vi "VIH Dialog - VI Terminals - Conpane Image.vi"(8 "error in":errorcluster, 9 "Conpane Image":T1, 10 "Original VI Name":string, 11 "VI Reference":refnum<vi>) -> (0 "error out":errorcluster, 1 "Rectangle":T2, 2 "image":picture, 3 "dup VI Reference":refnum<vi>)   [LabVIEW 2014]
doc: "::: VI Helpeks :::\nCopyright (c) 2000-2026 Konstantin Shifershteyn. All rights reserved."
uses:
  <vilib>/picture/picture.llb/imagedata.ctl
  <vilib>/Utility/miscctls.llb/LVPointTypeDef.ctl
panel:
  in  "Default Image":picture
  in  "Font prototype":string
  # "VI Helpeks\nCopyright (c) 2012-2026 Konstantin Shifershteyn"
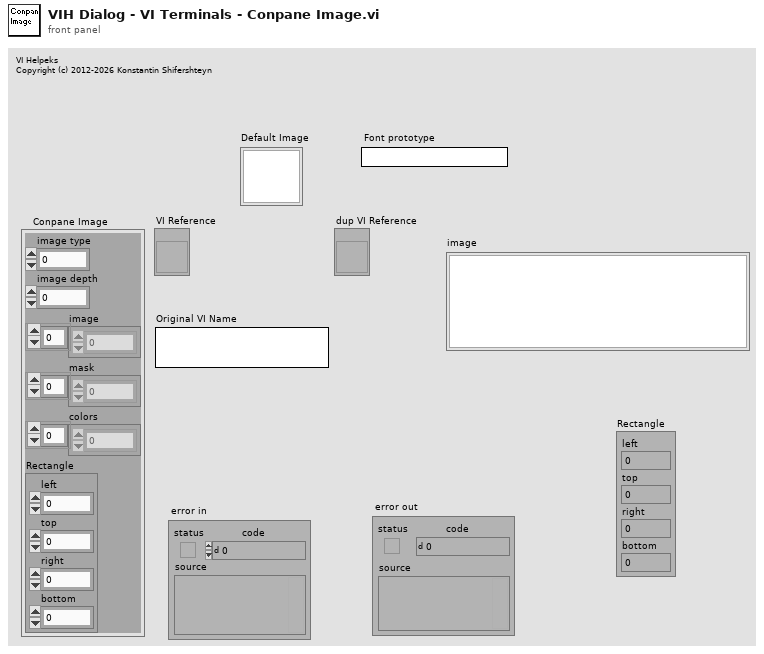
[diagram p1: front panel]
types:
  T1 = typedef "imagedata.ctl" = cluster{"image type":i32, "image depth":i32, "image":u8[], "mask":u8[], "colors":u32[], "Rectangle":cluster{"left":i16, "top":i16, "right":i16, "bottom":i16}}
  T2 = cluster{"left":i16, "top":i16, "right":i16, "bottom":i16}
  T3 = cluster{"Width":i16, "Style":enum32{"Solid", "Dash", "Dot", "DashDot", "DashDotDot"}}
  T4 = cluster{"Width":u16, "Style":enum32{"Solid", "Dash", "Dot", "DashDot", "DashDotDot"}}
  T5 = cluster{"Font Name:":string, "Size":i16, "Strikeout?":bool, "Italic?":bool, "Underline?":bool, "Outline?":bool, "Shadow?":bool, "Bold?":bool}
  T6 = enum16{"User-specified Font", "Application Font", "System Font", "Dialog Font"}
  T7 = typedef "LVPointTypeDef.ctl" = cluster{"Horizontal":i16, "Vertical":i16}
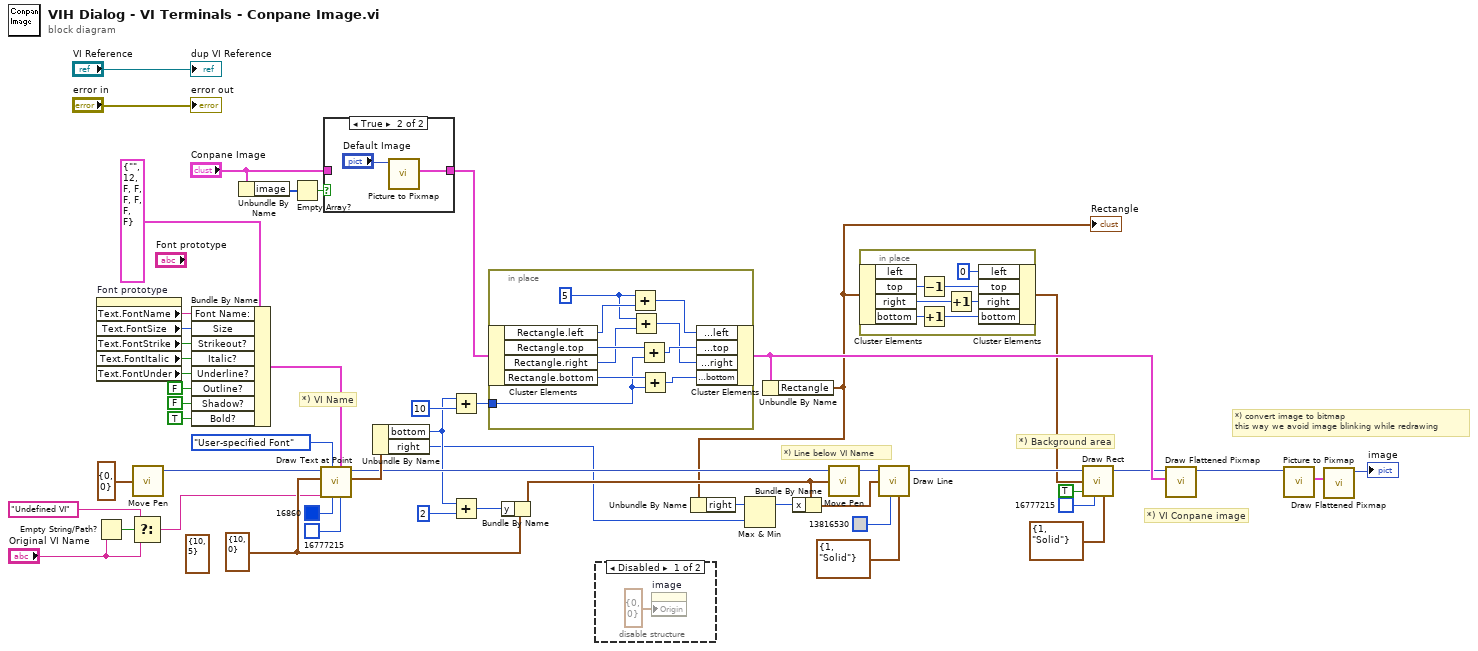
[diagram p0: block diagram]
diagram:
  (unwired) cluster{"x":i16, "y":i16} {"x"=10, "y"=5} ("origin")
  w24 = cluster{"x":i16, "y":i16} {"x"=10, "y"=0} ("origin")
  # "*) Background area"
  # "*) convert image to bitmap\nthis way we avoid image blinking while redrawing"
  # "*) VI Name"
  # "*) Line below VI Name"
  # "*) VI Conpane image"
  n1 = Empty String/Path?(string/path="Original VI Name") -> (empty?=w7:bool)
  n2 = property on="Font prototype" class="Str"() -> ("Text.FontName"=w41:string, "Text.FontSize"=w42:u32, "Text.FontStrike"=w43:bool, "Text.FontItalic"=w44:bool, "Text.FontUnder"=w45:bool)  [unwired: 2 in, 2 out]
  n3 = Select(t="Undefined VI", s=w7, f="Original VI Name") -> (s? t:f=w5:string)
  n4 = call <vilib>:"Move Pen.vi"("new position"=cluster{"x":i16, "y":i16} {"x"=0, "y"=0} ("origin")) -> ("new picture"=w19:picture)  [unwired: 4 in]
  n5 = Bundle By Name(cluster=T5 {"Font Name:"="", "Size"=12, "Strikeout?"=FALSE, "Italic?"=FALSE, "Underline?"=FALSE, "Outline?"=FALSE, "Shadow?"=FALSE, "Bold?"=FALSE} ("[user-specified font]"), "Font Name:"=w41, "Size"=w42, "Strikeout?"=w43, "Italic?"=w44, "Underline?"=w45, "Outline?"=FALSE, "Shadow?"=FALSE, "Bold?"=TRUE) -> (w39:T5)
  n6 = Unbundle By Name("Conpane Image") -> ("image"=w4:u8[])
  n7 = Empty Array?(array=w4) -> (empty?=w1:bool)
  n8 = call <vilib>:"Draw Text at Point.vi"("BG color(transparent)"=u32 16777215, "[user-specified font]"=w39, "text color(black)"=u32 16860, "desired font(Application)"=T6."User-specified Font", "text"=w5, "origin"=w24, "picture"=w19) -> ("text rect"=w52:T2, "new picture"=w32:picture)  [unwired: 3 in]
  n9 = case shown="True" w1 {
    tunnel: [w53 w54] -> w2
    tunnel: "Conpane Image" -> [w53 _]
    frame False {
    }
    frame True {
      n10 = call <vilib>:"Picture to Pixmap.vi"("picture"="Default Image") -> ("image data"=w54:T1)  [unwired: 9 in, 1 out]
    }
  }
  n11 = Unbundle By Name(w52) -> ("bottom"=w31:i16, "right"=w23:i16)
  n12 = Add(x=w31, y=i16 10) -> (x+y=w50:i16)
  n13 = Add(x=w31, y=i16 2) -> (x+y=w30:i16)
  n14 = in-place {
    in-place-border: w50 -> [w61]
    w58 = i16 5 ("x")
    n15 = in-place-cluster #1(w2) -> ("Rectangle.left"=w60:i16, "Rectangle.top"=w65:i16, "Rectangle.right"=w59:i16, "Rectangle.bottom"=w63:i16)
    n16 = Add(x=w58, y=w60) -> (x+y=w57:i16)
    n17 = Add(x=w58, y=w59) -> (x+y=w56:i16)
    n18 = Add(x=w65, y=w61) -> (x+y=w64:i16)
    n19 = Add(x=w63, y=w61) -> (x+y=w62:i16)
    n20 = in-place-cluster #1("Rectangle.left"=w57, "Rectangle.top"=w64, "Rectangle.right"=w56, "Rectangle.bottom"=w62) -> (w35:T1)
  }
  n21 = Bundle By Name(cluster=w24, "y"=w30) -> (w29:cluster{"x":i16, "y":i16})
  n22 = disable-structure shown="Disabled" {
    frame Disabled {
      n23 = property on="image" class="Pict"("Origin"=T7 {"Horizontal"=0, "Vertical"=0}) -> ()  [unwired: 2 in, 2 out]
    }
    frame Enabled {
    }
  }
  n24 = Unbundle By Name(w35) -> ("Rectangle"=w16:T2)
  "Rectangle" <- w16
  n25 = Unbundle By Name(w16) -> ("right"=w22:i16)
  n26 = Max & Min(x=w22, y=w23) -> (max(x,y)=w21:i16)  [unwired: 1 out]
  n27 = Bundle By Name(cluster=w29, "x"=w21) -> (w28:cluster{"x":i16, "y":i16})
  n28 = call <vilib>:"Move Pen.vi"("new position"=w29, "picture"=w32) -> ("new picture"=w34:picture)  [unwired: 3 in]
  n29 = in-place {
    n30 = in-place-cluster #2(w16) -> ("top"=w69:i16, "right"=w73:i16, "bottom"=w71:i16)  [unwired: 1 out]
    n31 = Decrement(x=w69) -> (x-1=w68:i16)
    n32 = Increment(x=w71) -> (x+1=w70:i16)
    n33 = Increment(x=w73) -> (x+1=w72:i16)
    n34 = in-place-cluster #2("left"=i16 0, "top"=w68, "right"=w72, "bottom"=w70) -> (w15:T2)
  }
  n35 = call <vilib>:"Draw Line.vi"("picture"=w34, "end point"=w28, "color(black)"=u32 13816530, "pen"=T4 {"Width"=1, "Style"=enum."Solid"}) -> ("new picture"=w18:picture)  [unwired: 5 in]
  n36 = call <vilib>:"Draw Rect.vi"("picture"=w18, "rect"=w15, "fill?(F)"=TRUE, "color(black)"=u32 16777215, "pen"=T3 {"Width"=1, "Style"=enum."Solid"}) -> ("new picture"=w17:picture)  [unwired: 4 in]
  n37 = call <vilib>:"Draw Flattened Pixmap.vi"("image data"=w35, "picture"=w17) -> ("new picture"=w13:picture)  [unwired: 7 in]
  n38 = call <vilib>:"Picture to Pixmap.vi"("picture"=w13) -> ("image data"=w14:T1)  [unwired: 9 in, 1 out]
  n39 = call <vilib>:"Draw Flattened Pixmap.vi"("image data"=w14) -> ("new picture"=→"image":picture)  [unwired: 8 in]
  "error out" <- "error in"
  "dup VI Reference" <- "VI Reference"
